vi "Bounds.vi"(1 "XRef":refnum<vi>, 2 "State In":T2) -> (0 "Bounds":cluster{"Width":T1, "Height":T1})   [LabVIEW 2012, in "OpenG Index Array Element.xnode"]
uses:
  OpenG Index Array Element.xnode
  State.ctl
  <vilib>/XNodeSupport/XNodeInt.ctl
  <vilib>/XNodeSupport/NI_XNodeSupport.lvlib
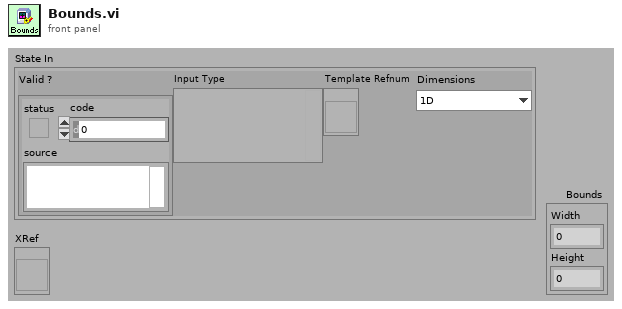
[diagram p1: front panel]
types:
  T1 = typedef "NI_XNodeSupport.lvlib/XNodeInt.ctl" = i32
  T2 = typedef "OpenG Index Array Element.xnode/State.ctl" = cluster{"Valid ?":errorcluster, "Input Type":variant, "Template Refnum":refnum<vi>, "Dimensions":enum16{"1D", "2D"}}
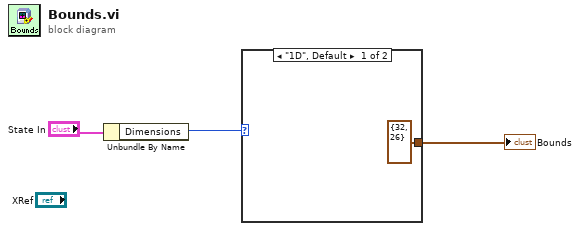
[diagram p0: block diagram]
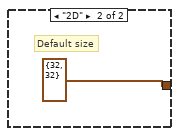
[diagram p2: hidden frame]
diagram:
  n1 = Unbundle By Name("State In") -> ("Dimensions"=w1:enum16{"1D", "2D"})
  n2 = case shown="\"1D\", Default" w1 {
    tunnel: [cluster{"Width":T1, "Height":T1} {"Width"=32, "Height"=26} ("Bounds") cluster{"Width":T1, "Height":T1} {"Width"=32, "Height"=32} ("Bounds")] -> w3
    frame "1D", Default {
    }
    frame "2D" {
      # "Default size"
    }
  }
  "Bounds" <- w3
